vi "DAQ_Engine.vi"(11 "error in":errorcluster) -> (15 "error out":errorcluster)   [LabVIEW 2026]
doc: "DAQ 엔진: 이름 있는 큐 AIDAQ_CMD 로 명령(Start/Stop/Config/Log On/Log Off/Exit)을 받아 128채널 측정.\n측정 데이터는 AIDAQ_LIVE(메인 화면), AIDAQ_GRAPH(그래프 팝업) 큐(크기 1, 최신값)로 보낸다. Exit 명령에 끝난다."
uses:
  <vilib>/DAQmx/miscellaneous.llb/DAQmx Fill In Error Info.vi
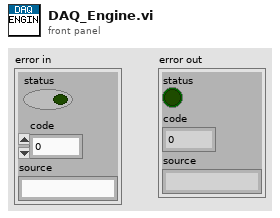
[diagram p1: front panel]
types:
  T1 = cluster{"Name":string, "Value":dbl, "High Limit":dbl, "Low Limit":dbl, "Save":bool, "Graph":bool, "Scale Min":dbl, "Scale Max":dbl, "Unit":string}[]
  T2 = cluster{"Data":dbl[][], "Values":dbl[], "dt":dbl, "Running":bool, "Logging":bool, "Message":string, "Log File":path}
  T3 = cluster{"Cmd":enum16{"Start", "Stop", "Config", "Log On", "Log Off", "Exit"}, "Settings":cluster{"Sample Rate (Hz)":dbl, "Samples per Channel":i32, "Chassis 1 Channels":string, "Chassis 2 Channels":string, "Save Folder":path}, "Channels":cluster{"Name":string, "Value":dbl, "High Limit":dbl, "Low Limit":dbl, "Save":bool, "Graph":bool, "Scale Min":dbl, "Scale Max":dbl, "Unit":string}[]}
  T4 = enum16{"Start", "Stop", "Config", "Log On", "Log Off", "Exit"}
  T5 = cluster{"Sample Rate (Hz)":dbl, "Samples per Channel":i32, "Chassis 1 Channels":string, "Chassis 2 Channels":string, "Save Folder":path}
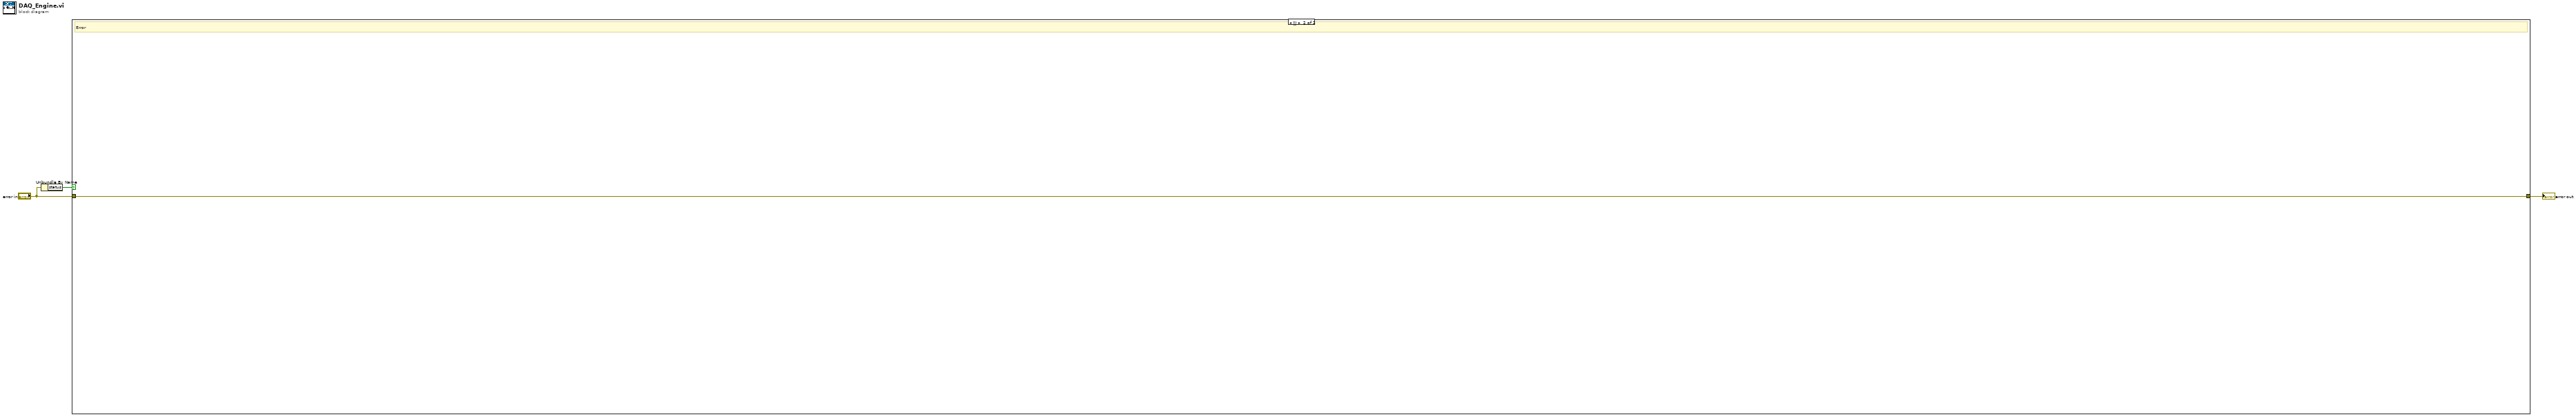
[diagram p0: block diagram]
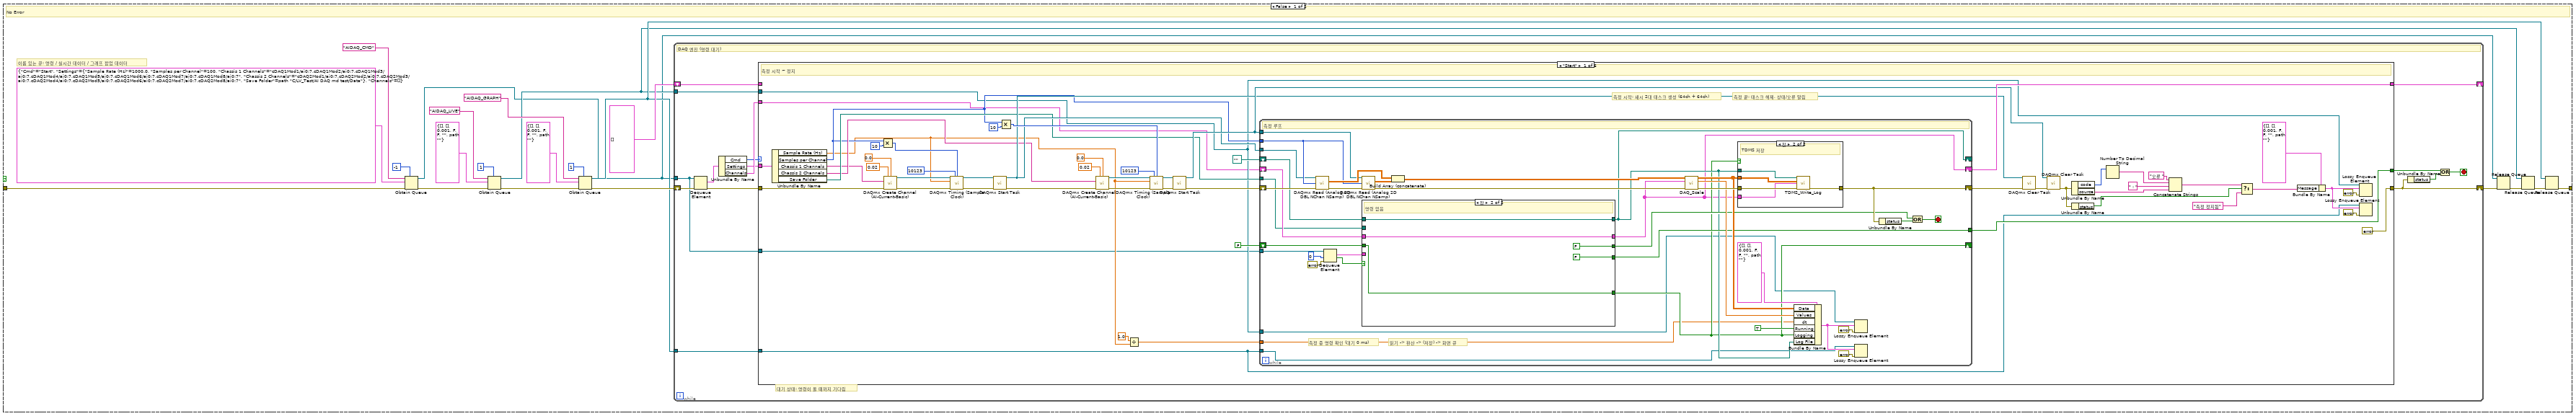
[diagram p2: hidden frame]
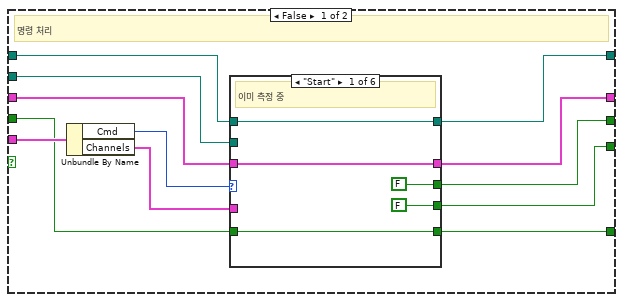
[diagram p4: hidden frame]
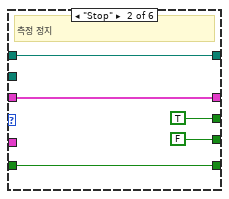
[diagram p5: hidden frame]
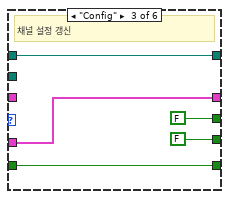
[diagram p6: hidden frame]
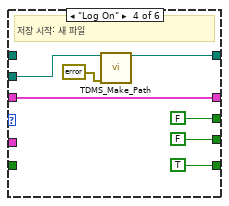
[diagram p7: hidden frame]
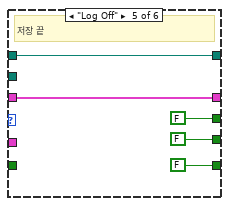
[diagram p8: hidden frame]
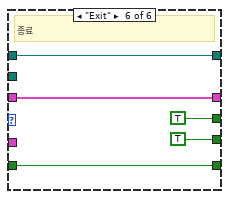
[diagram p9: hidden frame]
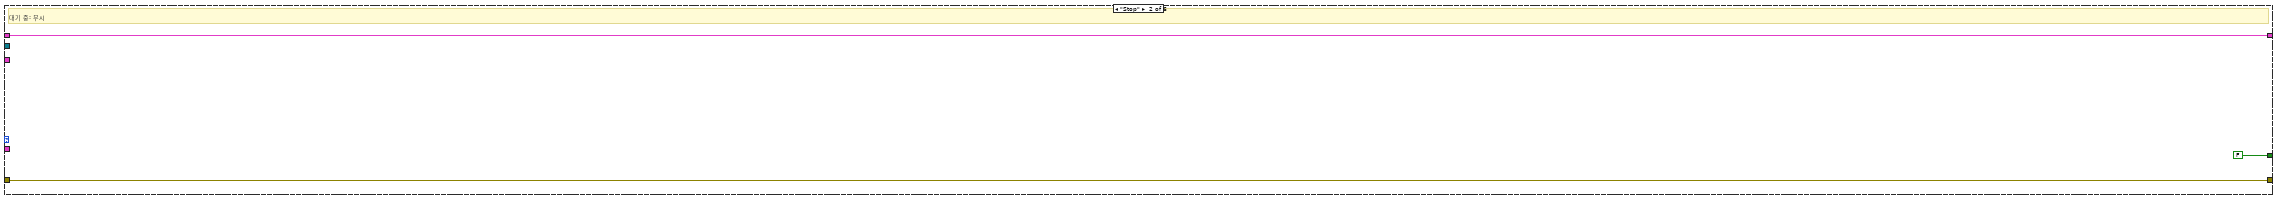
[diagram p10: hidden frame]
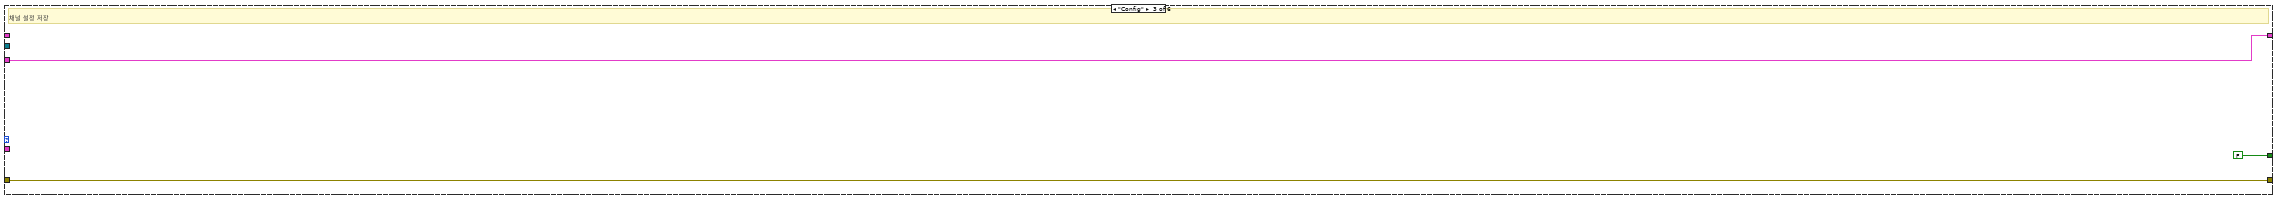
[diagram p11: hidden frame]
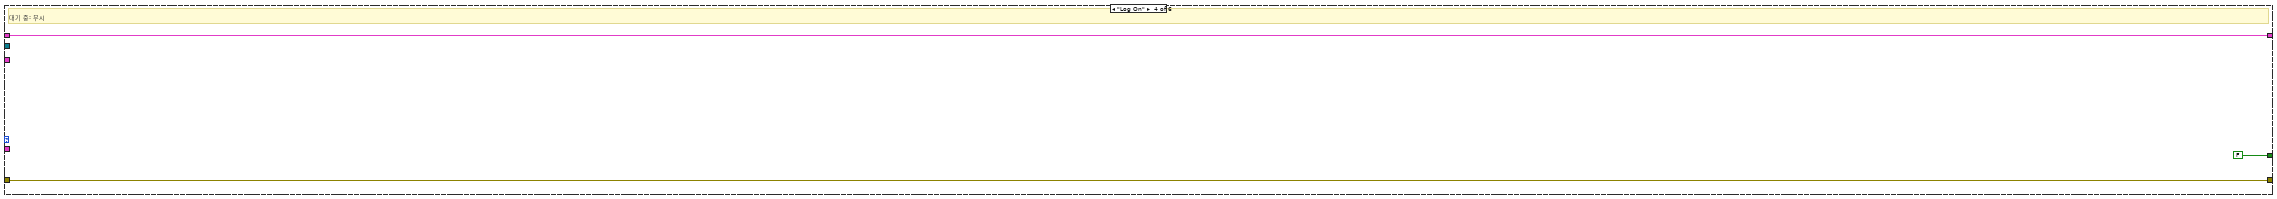
[diagram p12: hidden frame]
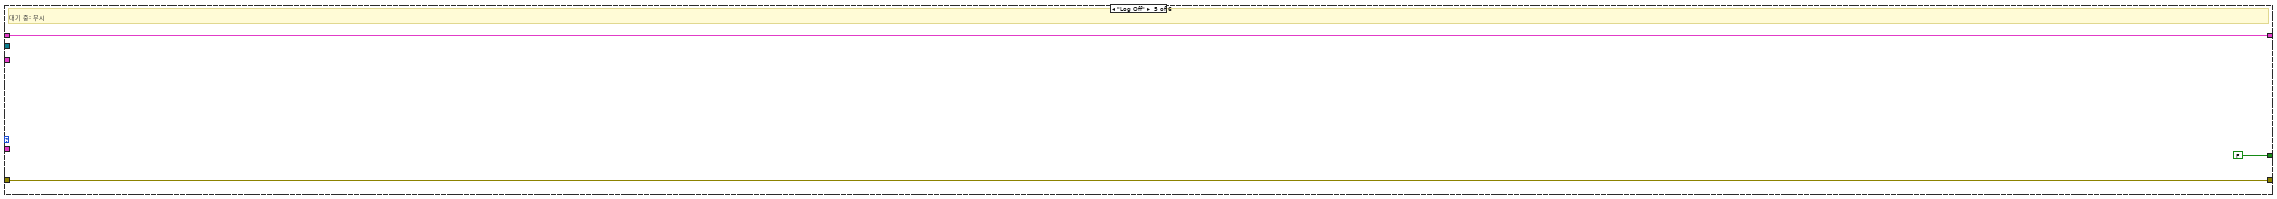
[diagram p13: hidden frame]
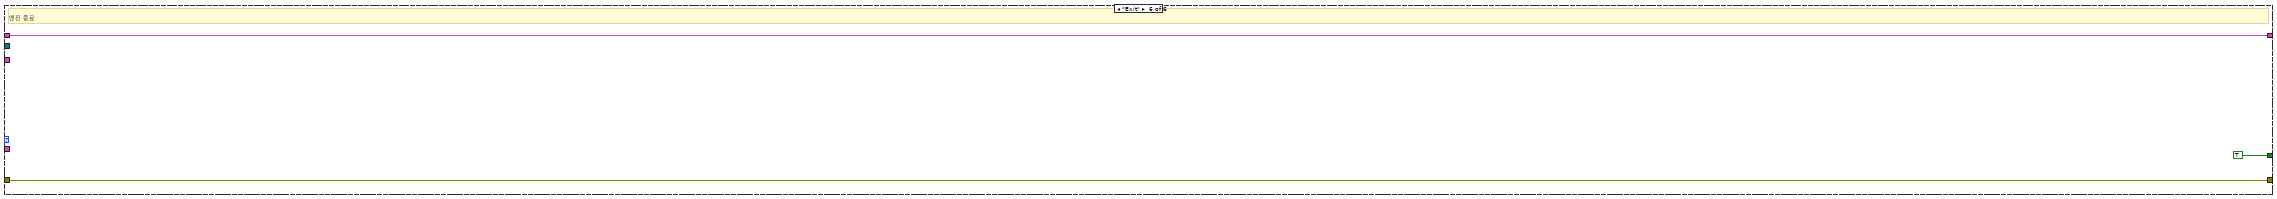
[diagram p14: hidden frame]
diagram:
  n1 = Unbundle By Name("error in") -> ("status"=w2:bool)
  n2 = case shown="참" w2 {
    tunnel: "error in" -> [w4 w203]
    tunnel: [w24 w203] -> w3
    frame False {
      # "이름 있는 큐: 명령 / 실시간 데이터 / 그래프 팝업 데이터"
      # "No Error"
      n3 = Obtain Queue(max queue size (-1, unlimited)=-1, name (unnamed)="AIDAQ_CMD", element data type=T3 {"Cmd"=enum."Start", "Settings"={"Sample Rate (Hz)"=1000.0, "Samples per Channel"=100, "Chassis 1 Channels"="cDAQ1Mod1/ai0:7,cDAQ1Mod2/ai0:7,cDAQ1Mod3/ai0:7,cDAQ1Mod4/ai0:7,cDAQ1Mod5/ai0:7,cDAQ1Mod6/ai0:7,cDAQ1Mod7/ai0:7,cDAQ1Mod8/ai0:7", "Chassis 2 Channels"="cDAQ2Mod1/ai0:7,cDAQ2Mod2/ai0:7,cDAQ2Mod3/ai0:7,cDAQ2Mod4/ai0:7,cDAQ2Mod5/ai0:7,cDAQ2Mod6/ai0:7,cDAQ2Mod7/ai0:7,cDAQ2Mod8/ai0:7", "Save Folder"=path "C:/LV_Test/AI DAQ md test/Data"}, "Channels"=[]}, error in (no error)=w4) -> (queue out=w8:refnum<queue>, error out=w9:errorcluster)  [unwired: 1 in, 1 out]
      n4 = Obtain Queue(max queue size (-1, unlimited)=1, name (unnamed)="AIDAQ_LIVE", element data type=T2 {"Data"=[], "Values"=[], "dt"=0.001, "Running"=FALSE, "Logging"=FALSE, "Message"="", "Log File"=path ""}, error in (no error)=w9) -> (queue out=w13:refnum<queue>, error out=w14:errorcluster)  [unwired: 1 in, 1 out]
      n5 = Obtain Queue(max queue size (-1, unlimited)=1, name (unnamed)="AIDAQ_GRAPH", element data type=T2 {"Data"=[], "Values"=[], "dt"=0.001, "Running"=FALSE, "Logging"=FALSE, "Message"="", "Log File"=path ""}, error in (no error)=w14) -> (queue out=w18:refnum<queue>, error out=w19:errorcluster)  [unwired: 1 in, 1 out]
      n6 = while {
        shift-right: [w35] -> _
        shift-left: T1 [] -> [w34]
        tunnel: w8 -> [w25]
        tunnel: w13 -> [w26]
        tunnel: w18 -> [w27]
        shift-right: [w37] -> w21
        shift-left: w19 -> [w30]
        stop <- w39 stop-if-true
        # "대기 상태: 명령이 올 때까지 기다림"
        # "DAQ 엔진 (명령 대기)"
        n7 = Dequeue Element(queue=w25, error in (no error)=w30) -> (element=w28:T3, error out=w29:errorcluster)  [unwired: 1 in, 2 out]
        n8 = Unbundle By Name(w28) -> ("Cmd"=w31:T4, "Settings"=w32:T5, "Channels"=w33:T1)
        n9 = case shown="\"Start\"" w31 {
          tunnel: [errorcluster {"status"=FALSE, "code"=0, "source"=""} w189 w191 w195 w198 w201] -> w37
          tunnel: w34 -> [_ w188 _ w194 w197 w200]
          tunnel: [w77 FALSE FALSE FALSE FALSE TRUE] -> w36
          tunnel: w25 -> [w43 _ _ _ _ _]
          tunnel: w26 -> [w44 _ _ _ _ _]
          tunnel: w27 -> [w45 _ _ _ _ _]
          tunnel: w29 -> [w40 w189 w191 w195 w198 w201]
          tunnel: w32 -> [w41 _ _ _ _ _]
          tunnel: w33 -> [w42 _ w192 _ _ _]
          tunnel: [w78 w188 w192 w194 w197 w200] -> w35
          frame "Start" {
            # "측정 끝: 태스크 해제, 상태/오류 알림"
            # "측정 시작: 섀시 2대 태스크 생성 (64ch + 64ch)"
            # "측정 시작 ~ 정지"
            n10 = Unbundle By Name(w41) -> ("Sample Rate (Hz)"=w46:dbl, "Samples per Channel"=w47:i32, "Chassis 1 Channels"=w48:string, "Chassis 2 Channels"=w49:string, "Save Folder"=w50:path)
            n11 = Multiply(x=w47, y=10) -> (x*y=w57:i32)
            n12 = call <vilib>:"DAQmx Create Channel (AI-Current-Basic).vi"("maximum value"=0.02, "minimum value"=0.0, "physical channels"=w48, "error in"=w40) -> ("task out"=w53:refnum<k21>, "error out"=w54:errorcluster)  [unwired: 10 in]
            n13 = call <vilib>:"DAQmx Timing (Sample Clock).vi"("task/channels in"=w53, "sample mode"=10123, "samples per channel"=w57, "rate"=w46, "error in"=w54) -> ("task out"=w58:refnum<k21>, "error out"=w59:errorcluster)  [unwired: 9 in]
            n14 = call <vilib>:"DAQmx Start Task.vi"("task/channels in"=w58, "error in"=w59) -> ("task out"=w60:refnum<k21>, "error out"=w61:errorcluster)  [unwired: 12 in]
            n15 = Multiply(x=w47, y=10) -> (x*y=w68:i32)
            n16 = call <vilib>:"DAQmx Create Channel (AI-Current-Basic).vi"("maximum value"=0.02, "minimum value"=0.0, "physical channels"=w49, "error in"=w61) -> ("task out"=w64:refnum<k21>, "error out"=w65:errorcluster)  [unwired: 10 in]
            n17 = Divide(x=1.0, y=w46) -> (x/y=w74:dbl)
            n18 = call <vilib>:"DAQmx Timing (Sample Clock).vi"("task/channels in"=w64, "sample mode"=10123, "samples per channel"=w68, "rate"=w46, "error in"=w65) -> ("task out"=w69:refnum<k21>, "error out"=w70:errorcluster)  [unwired: 9 in]
            n19 = call <vilib>:"DAQmx Start Task.vi"("task/channels in"=w69, "error in"=w70) -> ("task out"=w71:refnum<k21>, "error out"=w72:errorcluster)  [unwired: 12 in]
            n20 = while {
              shift-right: [w112] -> _
              shift-left: FALSE -> [w109]
              shift-right: [w113] -> _
              shift-left: path "" -> [w110]
              tunnel: [w115] -> w77
              tunnel: w43 -> [w100]
              tunnel: w44 -> [w101]
              tunnel: w45 -> [w102]
              shift-right: [w111] -> w78
              shift-left: w42 -> [w108]
              tunnel: w47 -> [w98]
              tunnel: w50 -> [w103]
              tunnel: w74 -> [w99]
              tunnel: w60 -> [w96]
              tunnel: w71 -> [w97]
              shift-right: [w125] -> w79
              shift-left: w72 -> [w118]
              stop <- w132 stop-if-true
              # "읽기 -> 환산 -> (저장) -> 화면 큐"
              # "측정 중 명령 확인 (대기 0 ms)"
              # "측정 루프"
              n21 = call <vilib>:"DAQmx Read (Analog 2D DBL NChan NSamp).vi"("task/channels in"=w96, "number of samples per channel"=w98, "error in"=w118) -> ("data"=w116:dbl[][], "error out"=w117:errorcluster)  [unwired: 10 in, 1 out]
              n22 = Dequeue Element(queue=w100, timeout in ms (-1)=0, error in (no error)=errorcluster {"status"=FALSE, "code"=0, "source"=""}) -> (element=w106:T3, timed out?=w107:bool)  [unwired: 2 out]
              n23 = call <vilib>:"DAQmx Read (Analog 2D DBL NChan NSamp).vi"("task/channels in"=w97, "number of samples per channel"=w98, "error in"=w117) -> ("data"=w119:dbl[][], "error out"=w120:errorcluster)  [unwired: 10 in, 1 out]
              n24 = case shown="참" w107 {
                tunnel: [w149 FALSE] -> w114
                tunnel: [w150 FALSE] -> w115
                tunnel: w109 -> [w140 w184]
                tunnel: w110 -> [w141 w185]
                tunnel: [w147 w184] -> w112
                tunnel: [w148 w185] -> w113
                tunnel: w106 -> [w142 _]
                tunnel: w108 -> [w139 w183]
                tunnel: w103 -> [w143 _]
                tunnel: [w146 w183] -> w111
                frame False {
                  # "명령 처리"
                  n25 = Unbundle By Name(w142) -> ("Cmd"=w144:T4, "Channels"=w145:T1)
                  n26 = case shown="\"Start\"" w144 {
                    tunnel: [FALSE TRUE FALSE FALSE FALSE TRUE] -> w149
                    tunnel: [FALSE FALSE FALSE FALSE FALSE TRUE] -> w150
                    tunnel: w140 -> [w152 w157 w161 _ _ w179]
                    tunnel: w141 -> [w153 w158 w162 _ w174 w180]
                    tunnel: [w152 w157 w161 TRUE FALSE w179] -> w147
                    tunnel: [w153 w158 w162 w169 w174 w180] -> w148
                    tunnel: w145 -> [_ _ w163 _ _ _]
                    tunnel: w139 -> [w151 w156 _ w166 w173 w178]
                    tunnel: w143 -> [_ _ _ w167 _ _]
                    tunnel: [w151 w156 w163 w166 w173 w178] -> w146
                    frame "Start" {
                      # "이미 측정 중"
                    }
                    frame "Stop" {
                      # "측정 정지"
                    }
                    frame "Config" {
                      # "채널 설정 갱신"
                    }
                    frame "Log On" {
                      # "저장 시작: 새 파일"
                      n27 = call "TDMS_Make_Path.vi"("Save Folder"=w167, "error in"=errorcluster {"status"=FALSE, "code"=0, "source"=""}) -> ("File Path"=w169:path)  [unwired: 12 in, 1 out]
                    }
                    frame "Log Off" {
                      # "저장 끝"
                    }
                    frame "Exit" {
                      # "종료"
                    }
                  }
                }
                frame True {
                  # "명령 없음"
                }
              }
              n28 = Build Array (concatenate)(w116, w119) -> (w121:dbl[][])
              n29 = call "DAQ_Scale.vi"("Raw Data (A)"=w121, "Channels"=w111, "error in"=w120) -> ("Scaled Data"=w122:dbl[][], "Values"=w123:dbl[], "error out"=w124:errorcluster)  [unwired: 10 in]
              n30 = case shown="참" w112 {
                tunnel: w113 -> [_ w134]
                tunnel: w111 -> [_ w136]
                tunnel: w122 -> [_ w135]
                tunnel: w124 -> [w133 w137]
                tunnel: [w133 w138] -> w125
                frame False {
                  # "저장 안 함"
                }
                frame True {
                  # "TDMS 저장"
                  n31 = call "TDMS_Write_Log.vi"("File Path"=w134, "Scaled Data"=w135, "Channels"=w136, "error in"=w137) -> ("error out"=w138:errorcluster)  [unwired: 11 in]
                }
              }
              n32 = Bundle By Name(cluster=T2 {"Data"=[], "Values"=[], "dt"=0.001, "Running"=FALSE, "Logging"=FALSE, "Message"="", "Log File"=path ""}, "Data"=w122, "Values"=w123, "dt"=w99, "Running"=TRUE, "Logging"=w112, "Log File"=w113) -> (w128:T2)
              n33 = Lossy Enqueue Element(queue=w101, element=w128, error in (no error)=errorcluster {"status"=FALSE, "code"=0, "source"=""}) -> ()  [unwired: 4 out]
              n34 = Lossy Enqueue Element(queue=w102, element=w128, error in (no error)=errorcluster {"status"=FALSE, "code"=0, "source"=""}) -> ()  [unwired: 4 out]
              n35 = Unbundle By Name(w125) -> ("status"=w131:bool)
              n36 = Or(x=w114, y=w131) -> (x .or. y?=w132:bool)
            }
            n37 = call <vilib>:"DAQmx Clear Task.vi"("task in"=w60, "error in"=w79) -> ("error out"=w80:errorcluster)  [unwired: 13 in]
            n38 = call <vilib>:"DAQmx Clear Task.vi"("task in"=w71, "error in"=w80) -> ("error out"=w81:errorcluster)  [unwired: 13 in]
            n39 = Unbundle By Name(w81) -> ("code"=w83:i32, "source"=w84:string)
            n40 = Unbundle By Name(w81) -> ("status"=w82:bool)
            n41 = Number To Decimal String(number=w83) -> (decimal integer string=w85:string)  [unwired: 1 in]
            n42 = Concatenate Strings("오류 ", w85, " : ", w84) -> (w88:string)
            n43 = Select(t=w88, s=w82, f="측정 정지됨") -> (s? t:f=w90:string)
            n44 = Bundle By Name(cluster=T2 {"Data"=[], "Values"=[], "dt"=0.001, "Running"=FALSE, "Logging"=FALSE, "Message"="", "Log File"=path ""}, "Message"=w90) -> (w92:T2)
            n45 = Lossy Enqueue Element(queue=w44, element=w92, error in (no error)=errorcluster {"status"=FALSE, "code"=0, "source"=""}) -> ()  [unwired: 4 out]
            n46 = Lossy Enqueue Element(queue=w45, element=w92, error in (no error)=errorcluster {"status"=FALSE, "code"=0, "source"=""}) -> ()  [unwired: 4 out]
          }
          frame "Stop" {
            # "대기 중: 무시"
          }
          frame "Config" {
            # "채널 설정 저장"
          }
          frame "Log On" {
            # "대기 중: 무시"
          }
          frame "Log Off" {
            # "대기 중: 무시"
          }
          frame "Exit" {
            # "엔진 종료"
          }
        }
        n47 = Unbundle By Name(w37) -> ("status"=w38:bool)
        n48 = Or(x=w36, y=w38) -> (x .or. y?=w39:bool)
      }
      n49 = Release Queue(queue=w8, error in (no error)=w21) -> (error out=w22:errorcluster)  [unwired: 1 in, 2 out]
      n50 = Release Queue(queue=w13, error in (no error)=w22) -> (error out=w23:errorcluster)  [unwired: 1 in, 2 out]
      n51 = Release Queue(queue=w18, error in (no error)=w23) -> (error out=w24:errorcluster)  [unwired: 1 in, 2 out]
    }
    frame True {
      # "Error"
    }
  }
  "error out" <- w3
